vi "main.vi"() -> ()   [LabVIEW 2025]
uses:
  <vilib>/Python/Open Venv Python Session.vi
  <vilib>/addons/database/Connection.llb/DB Tools Open Connec (Path).vi
  <vilib>/addons/database/Connection.llb/Conn Execute.vi
  <vilib>/addons/database/Recordset.llb/Rec Destroy - Connection.vi
  <vilib>/addons/database/Recordset.llb/Rec Fetch Recordset Data (R).vi
  <vilib>/addons/database/NI_Database_API.lvlib
panel:
  in  "Tab Control":T1(tab)
  out "Table Control":string[][](table)
  in  "stop":bool
  out "Message":string
  out "RESULT":string
  in  "data base 3":bool
  in  "Intruments 3":bool
  in  "Settings Button 3":bool
  in  "Name Instruments":string(combo)
  out "Table Control 2":string[][](table)
  in  "Home Button 3":bool
  out "error out 3":errorcluster
  out "return value":bool
  out "RESULT":string
  in  "Settings Button":bool
  in  "Preferences Button":bool
  in  "Home Button":bool
  in  "Preferences Button 2":bool
  in  "Camera number":i32
  in  "Ai model":path
  in  "module path":path
  in  "Intruments":bool
  out "error out":errorcluster
  in  "Intruments 2":bool
  in  "Name":string(combo)
  out "error out 2":errorcluster
  in  "connection information":path
  in  "Home Button 2":bool
  in  "Settings Button 2":bool
  in  "Id":string
  in  "Save Button":bool
  in  "Cancel Button":bool
  out "Boolean":bool
  # "HOME"
  # "INSTRUMENTS TABLE"
  # "PYTHON CONFIG"
  # "DATA BASE CONFIG"
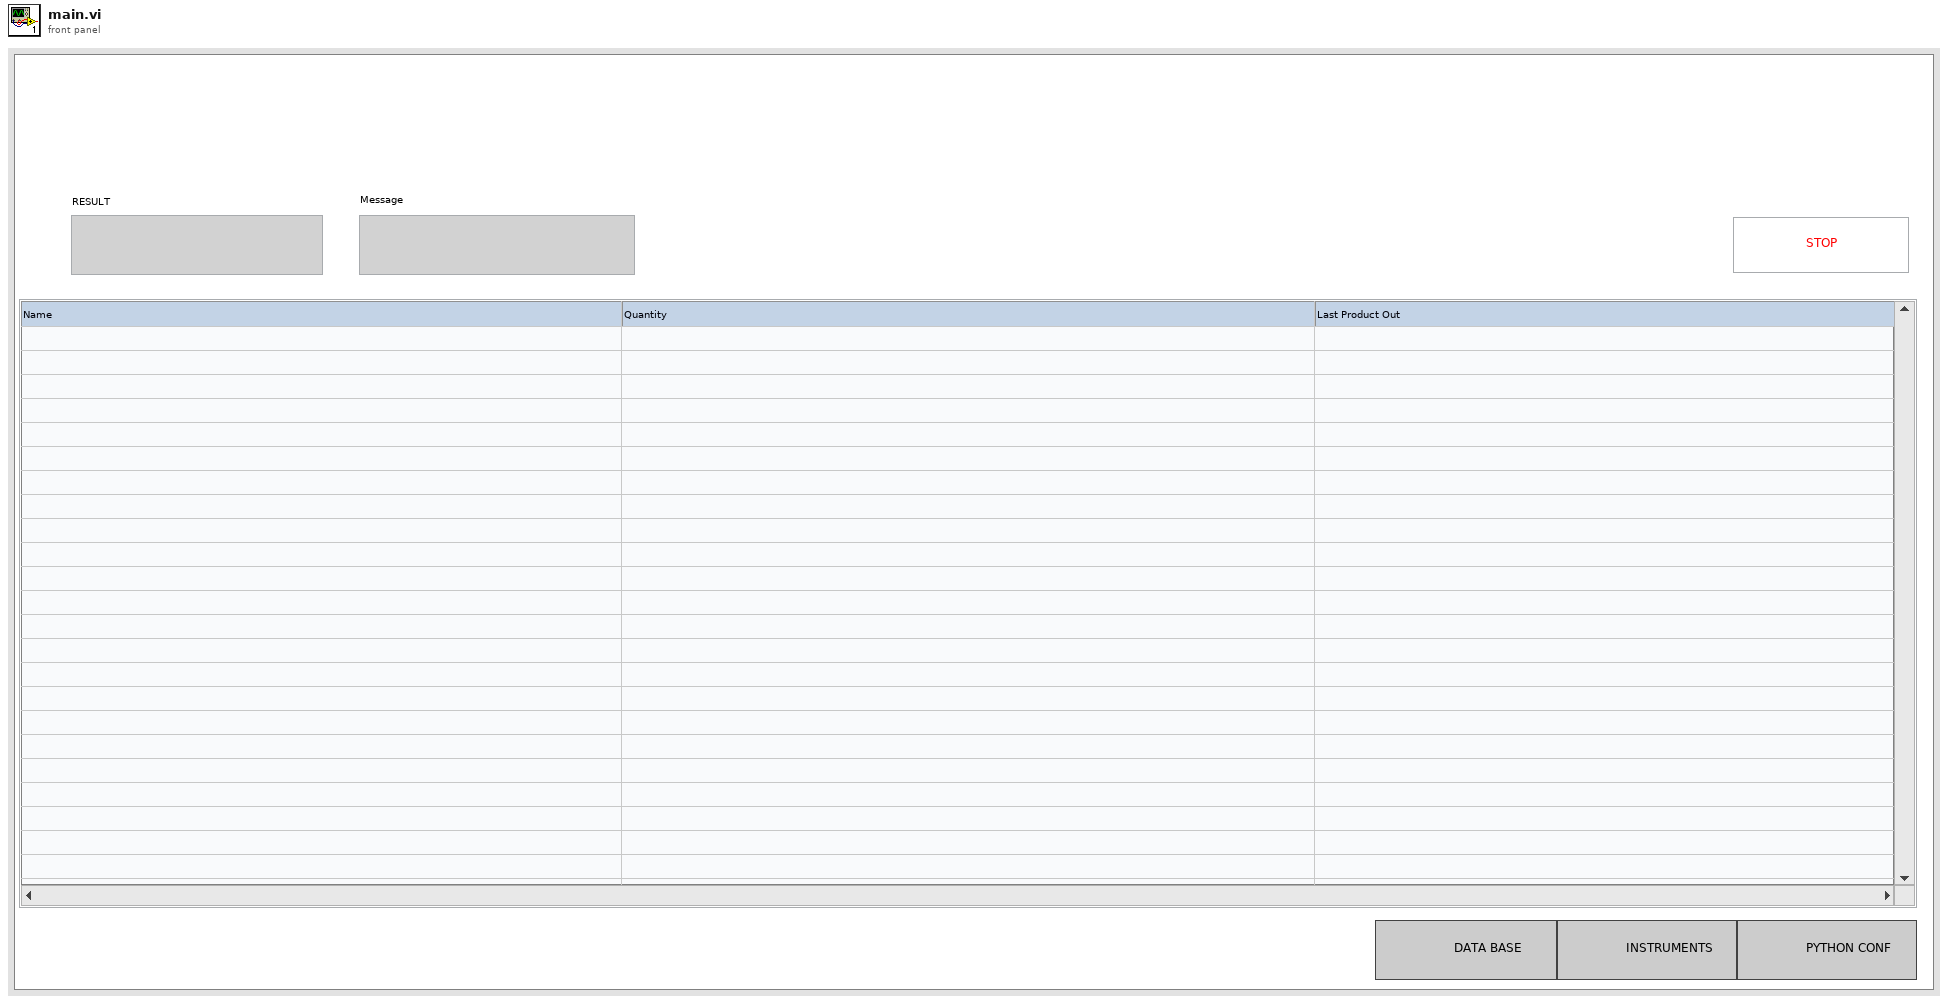
[diagram p1: front panel]
types:
  T1 = enum32{"Home", "INSTRUMENTS", "PYTHON CONFIG", "DATA BASE CONFIG"}
  T2 = typedef "NI_Database_API.lvlib/Conn ObjectReference.ctl" = refnum<k1>
  T3 = typedef "NI_Database_API.lvlib/Rec ObjectReference.ctl" = refnum<k1>
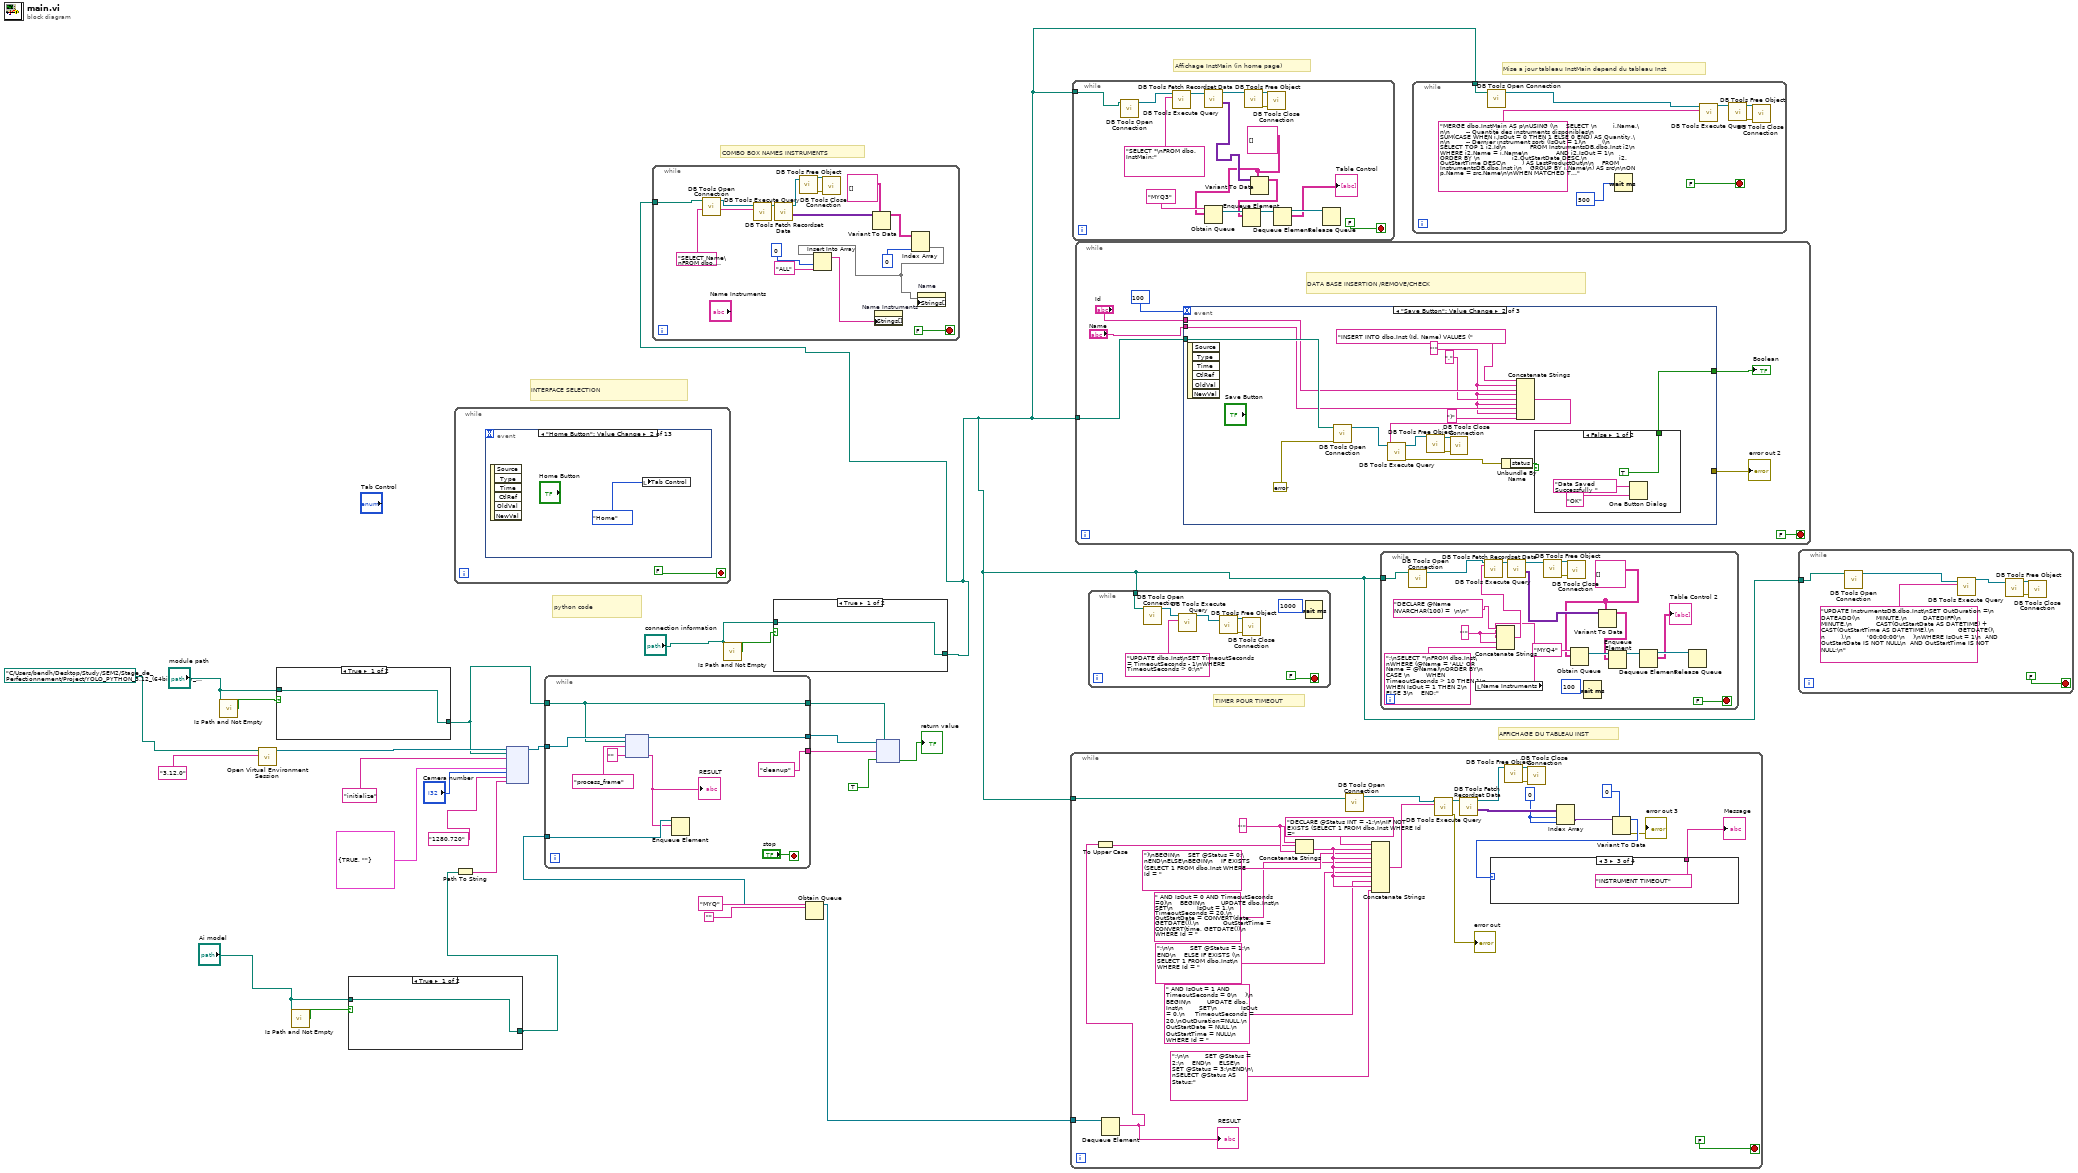
[diagram p0: block diagram]
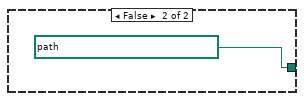
[diagram p2: hidden frame]
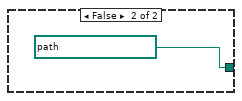
[diagram p3: hidden frame]
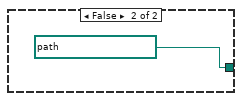
[diagram p4: hidden frame]
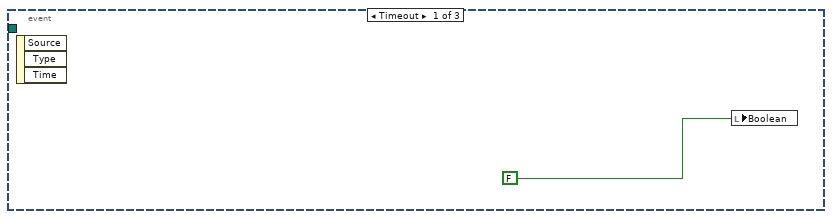
[diagram p5: hidden frame]
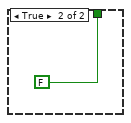
[diagram p6: hidden frame]
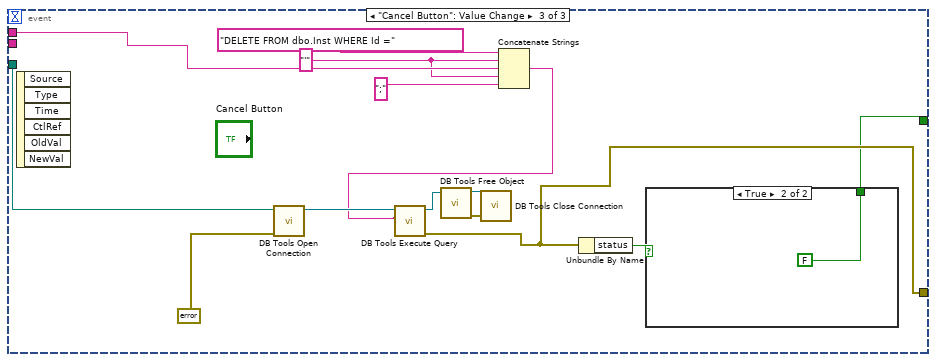
[diagram p7: hidden frame]
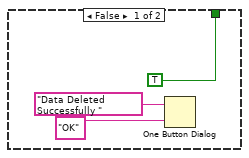
[diagram p8: hidden frame]
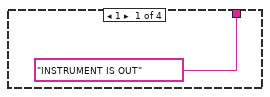
[diagram p9: hidden frame]
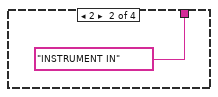
[diagram p10: hidden frame]
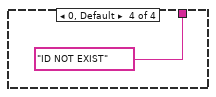
[diagram p11: hidden frame]
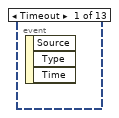
[diagram p12: hidden frame]
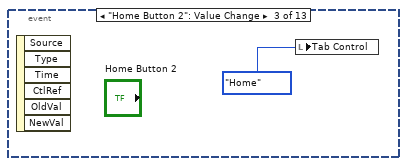
[diagram p13: hidden frame]
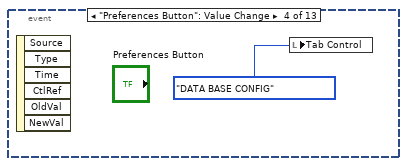
[diagram p14: hidden frame]
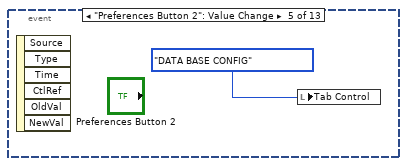
[diagram p15: hidden frame]
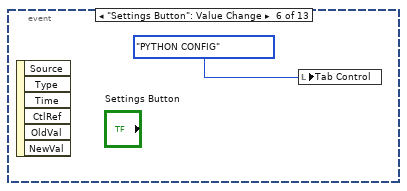
[diagram p16: hidden frame]
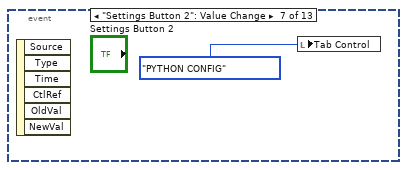
[diagram p17: hidden frame]
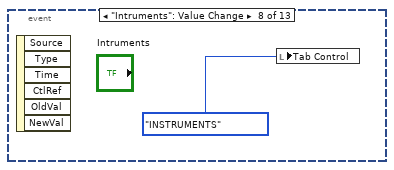
[diagram p18: hidden frame]
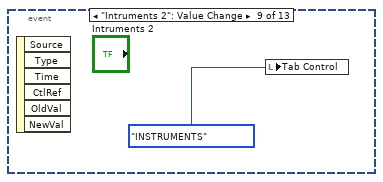
[diagram p19: hidden frame]
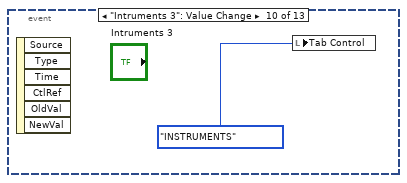
[diagram p20: hidden frame]
diagram:
  # "COMBO BOX NAMES INSTRUMENTS"
  # "Mise a jour tableau InstMain depend du tableau Inst"
  # "Affichage InstMain (in home page)"
  # "AFFICHAGE DU TABLEAU INST"
  # "TIMER POUR TIMEOUT"
  # "INTERFACE SELECTION"
  # "python code"
  n1 = call <vilib>:"Is Path and Not Empty.vi"("path"="module path") -> ("Is Path and Not Empty?"=w9:bool)  [unwired: 4 in]
  n2 = call-poly <vilib>:"Open Virtual Environment Session.vi"("Python version"="3.12.0", "Env path"=path "C:/Users/bendh/Desktop/Study/SEM2/Stage_de_Perfectionnement/Project/YOLO_PYTHON_3.12_(64bits)/venv_py312") -> ("session out"=w26:refnum<k35>)  [unwired: 8 in, 1 out]
  n3 = case shown="True" w9 {
    tunnel: [w27 path "C:/Users/bendh/Desktop/Study/SEM2/Stage_de_Perfectionnement/Project/LABVIEW/version opptimisé/app.py" ("module path")] -> w8
    tunnel: "module path" -> [w27 _]
    frame True {
    }
    frame False {
    }
  }
  n4 = call <vilib>:"Is Path and Not Empty.vi"("path"="Ai model") -> ("Is Path and Not Empty?"=w6:bool)  [unwired: 4 in]
  n5 = case shown="True" w6 {
    tunnel: [w29 path "C:/Users/bendh/Desktop/Study/SEM2/Stage_de_Perfectionnement/Project/LABVIEW/version opptimisé/my_model.pt" ("module path")] -> w4
    tunnel: "Ai model" -> [w29 _]
    frame True {
    }
    frame False {
    }
  }
  n6 = while {
    stop <- FALSE stop-if-true
    n7 = event shown="[1] \"Home Button\": Value Change" {
      selector: _ -> [_ _ _ _ _ _ _ _ _ _ _ _ _]
      dyn-events: _ -> [_ _ _ _ _ _ _ _ _ _ _ _ _]
      timeout: _ -> [_ _ _ _ _ _ _ _ _ _ _ _ _]
      event Timeout {
        n8 = event-data() -> ()  [unwired: 1 in, 3 out]
      }
      event "Home Button": Value Change {
        n9 = event-data() -> ()  [unwired: 1 in, 6 out]
        n10 = local write "Tab Control"(T1."Home" ("Tab Control 2")) -> ()
      }
      event "Home Button 2": Value Change {
        n11 = event-data() -> ()  [unwired: 1 in, 6 out]
        n12 = local write "Tab Control"(T1."Home" ("Tab Control 2")) -> ()
      }
      event "Preferences Button": Value Change {
        n13 = event-data() -> ()  [unwired: 1 in, 6 out]
        n14 = local write "Tab Control"(T1."DATA BASE CONFIG" ("Tab Control 2")) -> ()
      }
      event "Preferences Button 2": Value Change {
        n15 = event-data() -> ()  [unwired: 1 in, 6 out]
        n16 = local write "Tab Control"(T1."DATA BASE CONFIG" ("Tab Control 2")) -> ()
      }
      event "Settings Button": Value Change {
        n17 = event-data() -> ()  [unwired: 1 in, 6 out]
        n18 = local write "Tab Control"(T1."PYTHON CONFIG" ("Tab Control 2")) -> ()
      }
      event "Settings Button 2": Value Change {
        n19 = event-data() -> ()  [unwired: 1 in, 6 out]
        n20 = local write "Tab Control"(T1."PYTHON CONFIG" ("Tab Control 2")) -> ()
      }
      event "Intruments": Value Change {
        n21 = event-data() -> ()  [unwired: 1 in, 6 out]
        n22 = local write "Tab Control"(T1."INSTRUMENTS" ("Tab Control 2")) -> ()
      }
      event "Intruments 2": Value Change {
        n23 = event-data() -> ()  [unwired: 1 in, 6 out]
        n24 = local write "Tab Control"(T1."INSTRUMENTS" ("Tab Control 2")) -> ()
      }
      event "Intruments 3": Value Change {
        n25 = event-data() -> ()  [unwired: 1 in, 6 out]
        n26 = local write "Tab Control"(T1."INSTRUMENTS" ("Tab Control 2")) -> ()
      }
      event "Settings Button 3": Value Change {
        n27 = event-data() -> ()  [unwired: 1 in, 6 out]
        n28 = local write "Tab Control"(T1."PYTHON CONFIG" ("Tab Control 2")) -> ()
      }
      event "Home Button 3": Value Change {
        n29 = event-data() -> ()  [unwired: 1 in, 6 out]
        n30 = local write "Tab Control"(T1."Home" ("Tab Control 2")) -> ()
      }
      event "data base 3": Value Change {
        n31 = event-data() -> ()  [unwired: 1 in, 6 out]
        n32 = local write "Tab Control"(T1."DATA BASE CONFIG" ("Tab Control 2")) -> ()
      }
    }
  }
  n33 = Path To String(path=w4) -> (string=w23:string)
  n34 = node(w26, w8, "initialize" ("function name"), cluster{bool, string} {TRUE, ""}, "Camera number", "1280,720" ("input parameter"), w23) -> (w24:refnum<k35>)  [unwired: 5 in, 3 out]
  n35 = call <vilib>:"Is Path and Not Empty.vi"("path"="connection information") -> ("Is Path and Not Empty?"=w3:bool)  [unwired: 4 in]
  n36 = case shown="True" w3 {
    tunnel: [w44 path "C:/Users/bendh/Desktop/Study/SEM2/Stage_de_Perfectionnement/Project/LABVIEW/version opptimisé/SQL.udl" ("module path")] -> w1
    tunnel: "connection information" -> [w44 _]
    frame True {
    }
    frame False {
    }
  }
  n37 = while {
    tunnel: w1 -> [w60]
    stop <- FALSE stop-if-true
    n38 = call-poly <vilib>:"DB Tools Open Connection.vi"("connection information"=w60) -> ("connection reference"=w59:T2)  [unwired: 7 in, 1 out]
    n39 = call-poly <vilib>:"DB Tools Execute Query.vi"("SQL query"="SELECT Name\nFROM dbo.InstMain;", "connection reference"=w59) -> ("recordset reference"=w58:T3)  [unwired: 6 in, 1 out]
    n40 = call-poly <vilib>:"DB Tools Fetch Recordset Data.vi"("recordset reference"=w58) -> ("recordset data"=w57:variant[][], "recordset reference out"=w46:T3)  [unwired: 4 in, 1 out]
    n41 = call-poly <vilib>:"DB Tools Free Object.vi"("recordset reference"=w46) -> ("error out"=w48:errorcluster, "connection reference"=w47:T2)  [unwired: 9 in]
    n42 = call <vilib>:"DB Tools Close Connection.vi"("error in (no error)"=w48, "connection reference"=w47) -> ()  [unwired: 5 in, 1 out]
    n43 = Variant To Data(type=string[][] [] ("Array - String"), Variant=w57) -> (data=w55:string[][])  [unwired: 1 in, 1 out]
    n44 = Index Array(array=w55, index (col)=0) -> (element=w52:string[])  [unwired: 1 in]
    n45 = Insert Into Array(array=w52, index=0, new element="ALL" ("new element/subarray")) -> (w49:string[])
    n46 = property on="Name Instruments" class="CmbBox"("Strings[]"=w49) -> ()  [unwired: 2 in, 2 out]
    n47 = property on="Name" class="CmbBox"("Strings[]"=w52) -> ()  [unwired: 2 in, 2 out]
  }
  n48 = Obtain Queue(name (unnamed)="MYQ", element data type="") -> (queue out=w11:refnum<queue>)  [unwired: 3 in, 2 out]
  n49 = while {
    tunnel: w24 -> [w70]
    tunnel: w8 -> [w66]
    tunnel: [w67] -> w17
    tunnel: [w66] -> w16
    tunnel: w11 -> [w64]
    tunnel: ["cleanup" ("function name")] -> w10
    stop <- "stop" stop-if-true
    n50 = node(w70, w66, "process_frame" ("function name"), "") -> (w67:refnum<k35>, w63:string)  [unwired: 1 in, 3 out]
    "RESULT" <- w63
    n51 = Enqueue Element(queue=w64, element=w63) -> ()  [unwired: 2 in, 3 out]
  }
  n52 = node(w17, w16, w10, TRUE) -> (→"return value":bool)  [unwired: 1 in, 4 out]
  n53 = while {
    tunnel: w1 -> [w71]
    tunnel: w11 -> [w82]
    stop <- FALSE stop-if-true
    w86 = 0 ("index (row)")
    w94 = "'" ("string")
    n54 = Dequeue Element(queue=w82) -> (element=w81:string)  [unwired: 2 in, 3 out]
    "RESULT" <- w81
    n55 = To Upper Case(1:w81) -> (0:w84:string)
    n56 = Concatenate Strings(w94, w84, w94) -> (w97:string)
    n57 = call-poly <vilib>:"DB Tools Open Connection.vi"("connection information"=w71) -> ("connection reference"=w72:T2)  [unwired: 7 in, 1 out]
    n58 = Concatenate Strings("DECLARE @Status INT = -1;\n\nIF NOT EXISTS (SELECT 1 FROM dbo.Inst WHERE Id =" ("string"), w97, ")\nBEGIN\n    SET @Status = 0;\nEND\nELSE\nBEGIN\n    IF EXISTS (SELECT 1 FROM dbo.Inst WHERE Id = " ("string"), w97, " AND IsOut = 0 AND TimeoutSeconds =0)\n    BEGIN\n        UPDATE dbo.Inst\n        SET\n            IsOut = 1,\n            TimeoutSeconds = 20,\n            OutStartDate = CONVERT(date, GETDATE()),\n            OutStartTime = CONVERT(time, GETDATE())\n        WHERE Id = " ("string"), w97, ";\n\n        SET @Status = 1;\n    END\n    ELSE IF EXISTS (\n        SELECT 1 FROM dbo.Inst\n        WHERE Id = " ("string"), w97, " AND IsOut = 1 AND TimeoutSeconds = 0\n    )\n    BEGIN\n        UPDATE dbo.Inst\n        SET\n            IsOut = 0,\n     TimeoutSeconds = 20,\nOutDuration=NULL,\n            OutStartDate = NULL,\n            OutStartTime = NULL\n        WHERE Id = " ("string"), w97, ";\n\n        SET @Status = 2;\n    END\n    ELSE\n        SET @Status = 3;\nEND\n\nSELECT @Status AS Status;" ("string")) -> (w96:string)
    n59 = call-poly <vilib>:"DB Tools Execute Query.vi"("SQL query"=w96, "connection reference"=w72) -> ("error out"=→"error out":errorcluster, "recordset reference"=w95:T3)  [unwired: 6 in]
    n60 = call-poly <vilib>:"DB Tools Fetch Recordset Data.vi"("recordset reference"=w95) -> ("recordset data"=w87:variant[][], "recordset reference out"=w73:T3)  [unwired: 4 in, 1 out]
    n61 = call-poly <vilib>:"DB Tools Free Object.vi"("recordset reference"=w73) -> ("error out"=w75:errorcluster, "connection reference"=w74:T2)  [unwired: 9 in]
    n62 = call <vilib>:"DB Tools Close Connection.vi"("error in (no error)"=w75, "connection reference"=w74) -> ()  [unwired: 5 in, 1 out]
    n63 = Index Array(array=w87, index (row)=w86, index (col)=w86) -> (element=w80:variant)
    n64 = Variant To Data(type=0, Variant=w80) -> (data=w79:i32, error out=→"error out 3":errorcluster)  [unwired: 1 in]
    n65 = case shown="3" w79 {
      tunnel: ["INSTRUMENT IS OUT" ("String") "INSTRUMENT IN" ("String") "INSTRUMENT TIMEOUT" ("String") "ID NOT EXIST" ("String")] -> w85
      frame 1 {
      }
      frame 2 {
      }
      frame 3 {
      }
      frame 0, Default {
      }
    }
    "Message" <- w85
  }
  n66 = while {
    tunnel: w1 -> [w103]
    stop <- FALSE stop-if-true
    w107 = string[][] [] ("Array - String")
    n67 = call-poly <vilib>:"DB Tools Open Connection.vi"("connection information"=w103) -> ("connection reference"=w102:T2)  [unwired: 7 in, 1 out]
    n68 = call-poly <vilib>:"DB Tools Execute Query.vi"("SQL query"="SELECT *\nFROM dbo.InstMain;", "connection reference"=w102) -> ("recordset reference"=w115:T3)  [unwired: 6 in, 1 out]
    n69 = call-poly <vilib>:"DB Tools Fetch Recordset Data.vi"("recordset reference"=w115) -> ("recordset data"=w114:variant[][], "recordset reference out"=w104:T3)  [unwired: 4 in, 1 out]
    n70 = Obtain Queue(name (unnamed)="MYQ3", element data type=w107) -> (queue out=w111:refnum<queue>)  [unwired: 3 in, 2 out]
    n71 = call-poly <vilib>:"DB Tools Free Object.vi"("recordset reference"=w104) -> ("error out"=w106:errorcluster, "connection reference"=w105:T2)  [unwired: 9 in]
    n72 = Variant To Data(type=w107, Variant=w114) -> (data=w110:string[][])  [unwired: 1 in, 1 out]
    n73 = Enqueue Element(queue=w111, element=w110) -> (queue out=w112:refnum<queue>)  [unwired: 2 in, 2 out]
    n74 = call <vilib>:"DB Tools Close Connection.vi"("error in (no error)"=w106, "connection reference"=w105) -> ()  [unwired: 5 in, 1 out]
    n75 = Dequeue Element(queue=w112) -> (queue out=w113:refnum<queue>, element=→"Table Control":string[][])  [unwired: 2 in, 2 out]
    n76 = Release Queue(queue=w113) -> ()  [unwired: 2 in, 3 out]
  }
  n77 = while {
    tunnel: w1 -> [w120]
    stop <- FALSE stop-if-true
    # "DATA BASE INSERTION /REMOVE/CHECK"
    n78 = event shown="[1] \"Save Button\": Value Change" {
      selector: _ -> [_ _ _]
      dyn-events: _ -> [_ _ _]
      timeout: 100 -> [_ _ _]
      tunnel: w120 -> [_ w141 w159]
      tunnel: "Id" -> [_ w136 w155]
      tunnel: "Name" -> [_ w134 _]
      tunnel: [_ _ w150] -> w122
      tunnel: [_ w129 w149] -> w121
      event Timeout {
        n79 = event-data() -> ()  [unwired: 1 in, 3 out]
        n80 = local write "Boolean"(FALSE) -> ()
      }
      event "Save Button": Value Change {
        w133 = "'" ("string")
        n81 = event-data() -> ()  [unwired: 1 in, 6 out]
        n82 = call-poly <vilib>:"DB Tools Open Connection.vi"("error in (no error)"=errorcluster {"status"=FALSE, "code"=0, "source"=""}, "connection information"=w141) -> ("connection reference"=w139:T2)  [unwired: 6 in, 1 out]
        n83 = Concatenate Strings("INSERT INTO dbo.Inst (Id, Name) VALUES (", w133, w136, w133, "," ("string"), w133, w134, w133, ")" ("string")) -> (w138:string)
        n84 = call-poly <vilib>:"DB Tools Execute Query.vi"("SQL query"=w138, "connection reference"=w139) -> ("error out"=w131:errorcluster, "recordset reference"=w126:T3)  [unwired: 6 in]
        n85 = call-poly <vilib>:"DB Tools Free Object.vi"("recordset reference"=w126) -> ("error out"=w128:errorcluster, "connection reference"=w127:T2)  [unwired: 9 in]
        n86 = call <vilib>:"DB Tools Close Connection.vi"("error in (no error)"=w128, "connection reference"=w127) -> ()  [unwired: 5 in, 1 out]
        n87 = Unbundle By Name(w131) -> ("status"=w130:bool)
        n88 = case shown="False" w130 {
          tunnel: [TRUE FALSE] -> w129
          frame False {
            n89 = One Button Dialog(message="Data Saved Successfully ", button name ("OK")="OK") -> ()  [unwired: 1 out]
          }
          frame True {
          }
        }
      }
      event "Cancel Button": Value Change {
        w154 = "'" ("string")
        n90 = event-data() -> ()  [unwired: 1 in, 6 out]
        n91 = call-poly <vilib>:"DB Tools Open Connection.vi"("error in (no error)"=errorcluster {"status"=FALSE, "code"=0, "source"=""}, "connection information"=w159) -> ("connection reference"=w157:T2)  [unwired: 6 in, 1 out]
        n92 = Concatenate Strings("DELETE FROM dbo.Inst WHERE Id =" ("string"), w154, w155, w154, ";" ("string")) -> (w152:string)
        n93 = call-poly <vilib>:"DB Tools Execute Query.vi"("SQL query"=w152, "connection reference"=w157) -> ("error out"=w150:errorcluster, "recordset reference"=w146:T3)  [unwired: 6 in]
        n94 = call-poly <vilib>:"DB Tools Free Object.vi"("recordset reference"=w146) -> ("error out"=w148:errorcluster, "connection reference"=w147:T2)  [unwired: 9 in]
        n95 = call <vilib>:"DB Tools Close Connection.vi"("error in (no error)"=w148, "connection reference"=w147) -> ()  [unwired: 5 in, 1 out]
        n96 = Unbundle By Name(w150) -> ("status"=w151:bool)
        n97 = case shown="True" w151 {
          tunnel: [TRUE FALSE] -> w149
          frame False {
            n98 = One Button Dialog(message="Data Deleted Successfully ", button name ("OK")="OK") -> ()  [unwired: 1 out]
          }
          frame True {
          }
        }
      }
    }
    "error out 2" <- w122
    "Boolean" <- w121
  }
  n99 = while {
    tunnel: w1 -> [w164]
    stop <- FALSE stop-if-true
    n100 = call-poly <vilib>:"DB Tools Open Connection.vi"("connection information"=w164) -> ("connection reference"=w165:T2)  [unwired: 7 in, 1 out]
    n101 = call-poly <vilib>:"DB Tools Execute Query.vi"("SQL query"="UPDATE dbo.Inst\nSET TimeoutSeconds = TimeoutSeconds - 1\nWHERE TimeoutSeconds > 0;\n", "connection reference"=w165) -> ("recordset reference"=w166:T3)  [unwired: 6 in, 1 out]
    n102 = call-poly <vilib>:"DB Tools Free Object.vi"("recordset reference"=w166) -> ("error out"=w168:errorcluster, "connection reference"=w167:T2)  [unwired: 9 in]
    n103 = call <vilib>:"DB Tools Close Connection.vi"("error in (no error)"=w168, "connection reference"=w167) -> ()  [unwired: 5 in, 1 out]
    n104 = Wait (ms)(milliseconds to wait=u32 1000) -> ()  [unwired: 1 out]
  }
  n105 = while {
    tunnel: w1 -> [w173]
    stop <- FALSE stop-if-true
    w189 = "'" ("string")
    w176 = string[][] [] ("Array - String")
    n106 = call-poly <vilib>:"DB Tools Open Connection.vi"("connection information"=w173) -> ("connection reference"=w172:T2)  [unwired: 7 in, 1 out]
    n107 = local read "Name Instruments"() -> (w184:string)
    n108 = Concatenate Strings("DECLARE @Name NVARCHAR(100) =  \n\n" ("SQL query"), w189, w184, w189, ";\nSELECT *\nFROM dbo.Inst\nWHERE (@Name = 'ALL' OR Name = @Name)\nORDER BY\n    CASE \n        WHEN TimeoutSeconds > 10 THEN 1\n        WHEN IsOut = 1 THEN 2\n        ELSE 3\n    END;" ("string")) -> (w186:string)
    n109 = call-poly <vilib>:"DB Tools Execute Query.vi"("SQL query"=w186, "connection reference"=w172) -> ("recordset reference"=w192:T3)  [unwired: 6 in, 1 out]
    n110 = call-poly <vilib>:"DB Tools Fetch Recordset Data.vi"("recordset reference"=w192) -> ("recordset data"=w190:variant[][], "recordset reference out"=w181:T3)  [unwired: 4 in, 1 out]
    n111 = call-poly <vilib>:"DB Tools Free Object.vi"("recordset reference"=w181) -> ("error out"=w183:errorcluster, "connection reference"=w182:T2)  [unwired: 9 in]
    n112 = call <vilib>:"DB Tools Close Connection.vi"("error in (no error)"=w183, "connection reference"=w182) -> ()  [unwired: 5 in, 1 out]
    n113 = Obtain Queue(name (unnamed)="MYQ4", element data type=w176) -> (queue out=w178:refnum<queue>)  [unwired: 3 in, 2 out]
    n114 = Wait (ms)(milliseconds to wait=u32 100) -> ()  [unwired: 1 out]
    n115 = Variant To Data(type=w176, Variant=w190) -> (data=w175:string[][])  [unwired: 1 in, 1 out]
    n116 = Enqueue Element(queue=w178, element=w175) -> (queue out=w179:refnum<queue>)  [unwired: 2 in, 2 out]
    n117 = Dequeue Element(queue=w179) -> (queue out=w180:refnum<queue>, element=→"Table Control 2":string[][])  [unwired: 2 in, 2 out]
    n118 = Release Queue(queue=w180) -> ()  [unwired: 2 in, 3 out]
  }
  n119 = while {
    tunnel: w1 -> [w197]
    stop <- FALSE stop-if-true
    n120 = call-poly <vilib>:"DB Tools Open Connection.vi"("connection information"=w197) -> ("connection reference"=w196:T2)  [unwired: 7 in, 1 out]
    n121 = Wait (ms)(milliseconds to wait=u32 500) -> ()  [unwired: 1 out]
    n122 = call-poly <vilib>:"DB Tools Execute Query.vi"("SQL query"="MERGE dbo.InstMain AS p\nUSING (\n    SELECT \n        i.Name,\n\n        -- Quantité des instruments disponibles\n        SUM(CASE WHEN i.IsOut = 0 THEN 1 ELSE 0 END) AS Quantity,\n\n        -- Dernier instrument sorti (IsOut = 1)\n        (\n            SELECT TOP 1 i2.Id\n            FROM InstrumentsDB.dbo.Inst i2\n            WHERE i2.Name = i.Name\n              AND i2.IsOut = 1\n            ORDER BY \n                i2.OutStartDate DESC,\n                i2.OutStartTime DESC\n        ) AS LastProductOut\n\n    FROM InstrumentsDB.dbo.Inst i\n    GROUP BY i.Name\n) AS src\n\nON p.Name = src.Name\n\nWHEN MATCHED THEN\n    UPDATE SET \n        p.Quantity = src.Quantity,\n        p.LastProductOut = src.LastProductOut\n\nWHEN NOT MATCHED THEN\n    INSERT (Name, Quantity, LastProductOut)\n    VALUES (src.Name, src.Quantity, src.LastProductOut);\n", "connection reference"=w196) -> ("recordset reference"=w193:T3)  [unwired: 6 in, 1 out]
    n123 = call-poly <vilib>:"DB Tools Free Object.vi"("recordset reference"=w193) -> ("error out"=w195:errorcluster, "connection reference"=w194:T2)  [unwired: 9 in]
    n124 = call <vilib>:"DB Tools Close Connection.vi"("error in (no error)"=w195, "connection reference"=w194) -> ()  [unwired: 5 in, 1 out]
  }
  n125 = while {
    tunnel: w1 -> [w201]
    stop <- FALSE stop-if-true
    n126 = call-poly <vilib>:"DB Tools Open Connection.vi"("connection information"=w201) -> ("connection reference"=w202:T2)  [unwired: 7 in, 1 out]
    n127 = call-poly <vilib>:"DB Tools Execute Query.vi"("SQL query"="UPDATE InstrumentsDB.dbo.Inst\nSET OutDuration =\n    DATEADD(\n        MINUTE,\n        DATEDIFF(\n            MINUTE,\n            CAST(OutStartDate AS DATETIME) + CAST(OutStartTime AS DATETIME),\n            GETDATE()\n        ),\n        '00:00:00'\n    )\nWHERE IsOut = 1\n  AND OutStartDate IS NOT NULL\n  AND OutStartTime IS NOT NULL;\n", "connection reference"=w202) -> ("recordset reference"=w203:T3)  [unwired: 6 in, 1 out]
    n128 = call-poly <vilib>:"DB Tools Free Object.vi"("recordset reference"=w203) -> ("error out"=w205:errorcluster, "connection reference"=w204:T2)  [unwired: 9 in]
    n129 = call <vilib>:"DB Tools Close Connection.vi"("error in (no error)"=w205, "connection reference"=w204) -> ()  [unwired: 5 in, 1 out]
  }
